vi "SeqEditor_Name0Tip1ByData2.vi"(11 "output cluster":T1={"My"={"VIpath"={"ITEM"="VI路径", "DATA"="\"\"", "TYPE"=enum."Path", "TYPEDATA"="", "SV"=FALSE, "clusterchain"=[]}, "VIname"={"ITEM"="步骤名称", "DATA"="\"\"", "TYPE"=enum."String", "TYPEDATA"="", "SV"=FALSE, "clusterchain"=[]}, "Loop"={"ITEM"="重测次数", "DATA"="1", "TYPE"=enum."Number", "TYPEDATA"="", "SV"=FALSE, "clusterchain"=[]}, "Skip"={"ITEM"="跳过步骤", "DATA"="FALSE", "TYPE"=enum."Bool", "TYPEDATA"="", "SV"=FALSE, "clusterchain"=[]}, "FailStop"={"ITEM"="失败停止", "DATA"="FALSE", "TYPE"=enum."Bool", "TYPEDATA"="", "SV"=FALSE, "clusterchain"=[]}, "StepClass"={"ITEM"="步骤类型", "DATA"="NotaTEST", "TYPE"=enum."Enum", "TYPEDATA"="", "SV"=FALSE, "clusterchain"=[]}, "StringTest-Source"={"ITEM"="字符串测试值", "DATA"="\"\"", "TYPE"=enum."String", "TYPEDATA"="", "SV"=FALSE, "clusterchain"=[]}, "StringTest-Lim"={"ITEM"="字符串测试门限", "DATA"="\"\"", "TYPE"=enum."String", "TYPEDATA"="", "SV"=FALSE, "clusterchain"=[]}, "BoolTest-Source"={"ITEM"="布尔测试值", "DATA"="TRUE", "TYPE"=enum."Bool", "TYPEDATA"="", "SV"=FALSE, "clusterchain"=[]}, "BoolTest-Lim"={"ITEM"="布尔测试门限", "DATA"="TRUE", "TYPE"=enum."Bool", "TYPEDATA"="", "SV"=FALSE, "clusterchain"=[]}, "NumberTest-OP"={"ITEM"="数值测试OP", "DATA"="NotaTEST", "TYPE"=enum."Enum", "TYPEDATA"="", "SV"=FALSE, "clusterchain"=[]}, "NumberTest-Source"={"ITEM"="数值测试值", "DATA"="0", "TYPE"=enum."Number", "TYPEDATA"="", "SV"=FALSE, "clusterchain"=[]}, "NumberTest-LimA"={"ITEM"="数值测试门限A", "DATA"="0", "TYPE"=enum."Number", "TYPEDATA"="", "SV"=FALSE, "clusterchain"=[]}, "NumberTest-LimB"={"ITEM"="数值测试门限B", "DATA"="0", "TYPE"=enum."Number", "TYPEDATA"="", "SV"=FALSE, "clusterchain"=[]}}, "INPUT"=[], "OUTPUT"=[]}) -> (3 "Array":string[](array[string]))   [LabVIEW 2017, in "NLTest.lvclass"]
uses:
  NLTest.lvclass
  VISTEP.ctl
  VISTEP_class_INOUTPUT.ctl
  VISTEP_class_INOUTPUT_TYPE.ctl
panel:
  # "Y Y  LL"
types:
  T1 = typedef "NLTest.lvclass/VISTEP.ctl" = cluster{"My":cluster{"VIpath":T2, "VIname":T2, "Loop":T2, "Skip":T2, "FailStop":T2, "StepClass":T2, "StringTest-Source":T2, "StringTest-Lim":T2, "BoolTest-Source":T2, "BoolTest-Lim":T2, "NumberTest-OP":T2, "NumberTest-Source":T2, "NumberTest-LimA":T2, "NumberTest-LimB":T2}, "INPUT":T2[], "OUTPUT":T2[]}
  T2 = typedef "NLTest.lvclass/VISTEP_class_INOUTPUT.ctl" = cluster{"ITEM":string, "DATA":string, "TYPE":T3, "TYPEDATA":string, "SV":bool, "clusterchain":refnum<vi>[]}
  T3 = typedef "NLTest.lvclass/VISTEP_class_INOUTPUT_TYPE.ctl" = enum16{"Number", "String", "Bool", "Enum", "Path", "VISA", "NA"}
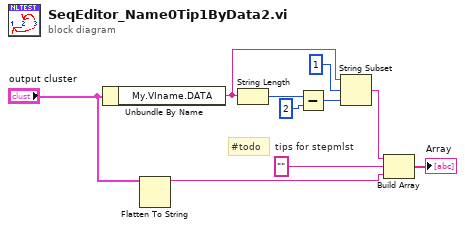
[diagram p0: block diagram]
diagram:
  w9 = ""  # tips for stepmlst
  # "#todo"
  n1 = Unbundle By Name("output cluster") -> ("My.VIname.DATA"=w2:string)
  n2 = Flatten To String(anything="output cluster") -> (data string=w10:string)  [unwired: 3 in, 2 out]
  n3 = String Length(string=w2) -> (length=w6:i32)
  n4 = Subtract(x=w6, y=2) -> (x-y=w4:i32)
  n5 = String Subset(string=w2, offset (0)=1, length (rest)=w4) -> (substring=w1:string)
  n6 = Build Array(w1, w9, w10) -> (→"Array":string[])
